vi "Right Click.vi"(6 "Empty Line?":bool, 7 "object refs":T2, 8 "error in (no error)":errorcluster, 9 "Coords":T1, 10 "Event data":variant, 11 "Multi Column Listbox in":refnum<class "Multi Column Listbox.lvclass">) -> (0 "error out":errorcluster, 3 "Multi Column Listbox out":refnum<class "Multi Column Listbox.lvclass">)   [LabVIEW 2014, in "Table Manager.lvlib" / "Multi Column Listbox.lvclass"]
doc: "Displays the menu options on a Right-Click."
uses:
  Multi Column Listbox.lvclass
  Table Manager/object ref.ctl
  Configuration Editor/Classes/Engine Parent/Engine Parent Editor Node.lvclass
  Configuration Editor/Classes/Module editor node/module editor node.lvclass
  <vilib>/Utility/miscctls.llb/LVPoint32TypeDef.ctl
  Multi Column Listbox.lvclass/Multi Column Listbox.ctl
  Table Manager/Menu Options.ctl
  <vilib>/NI/Tag Bus/tag/tag descriptor.lvclass
  Table Manager.lvlib
  <vilib>/NI/Tag Bus Module Framework/module configuration/TBM module configuration.lvclass
  Table Manager/Table Manager.lvclass
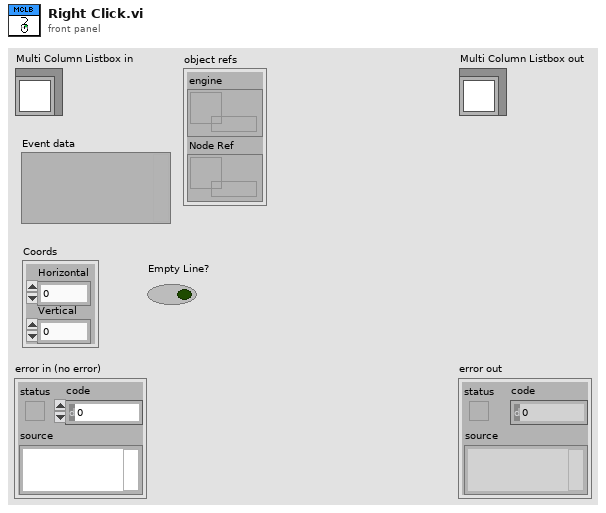
[diagram p1: front panel]
types:
  T1 = typedef "LVPoint32TypeDef.ctl" = cluster{"Horizontal":i32, "Vertical":i32}
  T2 = typedef "Table Manager.lvlib/Table Manager.lvclass/object ref.ctl" = cluster{"engine":refnum<data-value>, "Node Ref":refnum<data-value>}
  T3 = typedef "LVRowAndColumnTypeDef.ctl" = cluster{"Row":i32, "Column":i32}
  T4 = typedef "Table Manager.lvlib/Table Manager.lvclass/Menu Options.ctl" = enum16{"Always Show", "Show When Used", "Show When Empty"}
  T5 = typedef "Table Manager.lvlib/Table Manager.lvclass/Menu Definition.ctl" = cluster{"Menu Name":string, "Menu Options":T4}
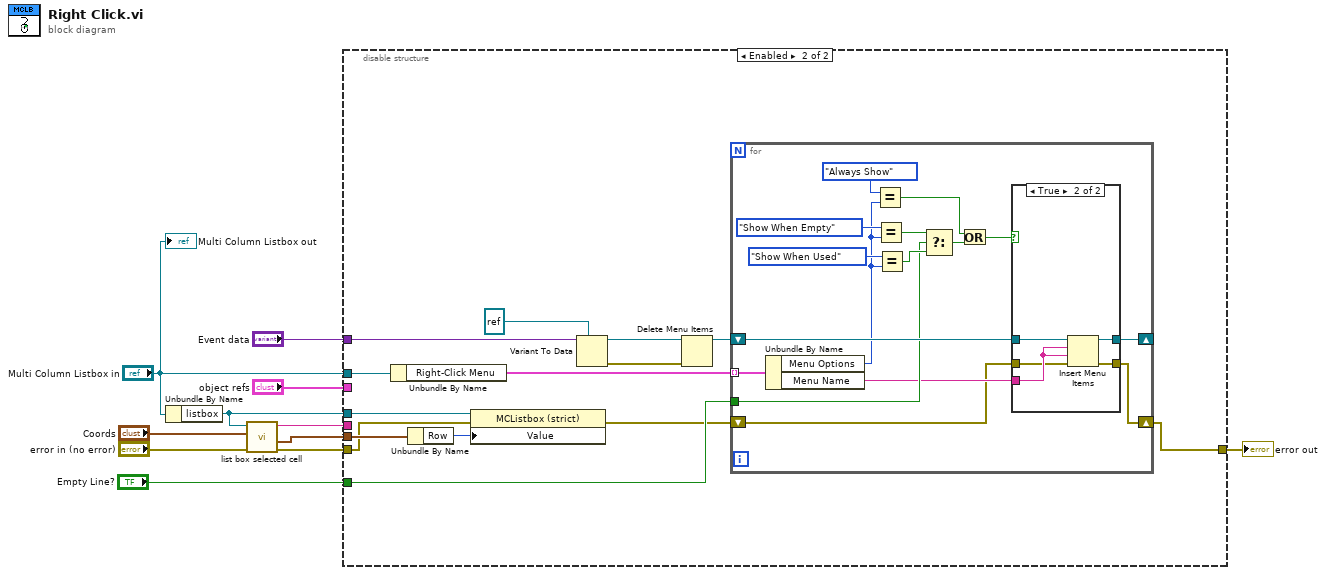
[diagram p0: block diagram]
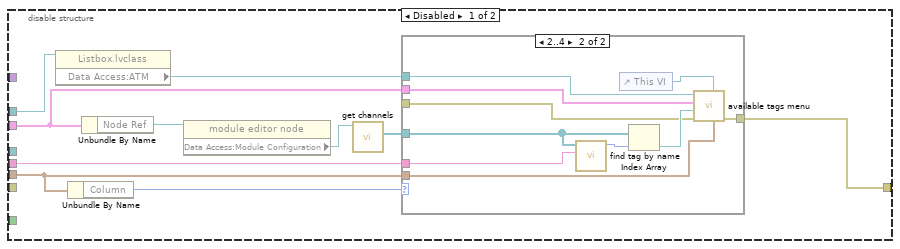
[diagram p2: hidden frame]
diagram:
  n1 = Unbundle By Name("Multi Column Listbox in") -> ("listbox"=w3:refnum<vi>)
  n2 = call "list box selected cell.vi"("error in"="error in (no error)", "Coords"="Coords", "MulticolumnListbox in"=w3) -> ("error out"=w5:errorcluster, "cell position"=w6:T3, "tag select name"=w7:string)  [unwired: 5 in, 1 out]
  n3 = disable-structure shown="Enabled" {
    disable-tunnel: "object refs" -> [w17 _]
    disable-tunnel: [w16 w33] -> w10
    disable-tunnel: "Multi Column Listbox in" -> [w15 w42]
    disable-tunnel: "Event data" -> [_ w46]
    disable-tunnel: w7 -> [w13 _]
    disable-tunnel: w6 -> [w12 w38]
    disable-tunnel: w5 -> [_ w35]
    disable-tunnel: w3 -> [_ w39]
    disable-tunnel: "Empty Line?" -> [_ w36]
    frame Disabled {
      n4 = property class="Listbox.lvclass"(reference=w15) -> ("Data Access:ATM"=w14:refnum<user-event>)  [unwired: 1 in, 2 out]
      n5 = Unbundle By Name(w12) -> ("Column"=w19:i32)
      n6 = Unbundle By Name(w17) -> ("Node Ref"=w18:refnum<data-value>)
      n7 = property class="module editor node"(reference=w18) -> ("Data Access:Module Configuration"=w21:refnum<class "TBM module configuration.lvclass">)  [unwired: 1 in, 2 out]
      n8 = call-dynamic "get channels.vi"("module configuration in"=w21) -> ("channels"=w20:refnum<class "TBM channel.lvclass">[])  [unwired: 9 in, 1 out]
      n9 = case shown="2..4" w19 {
        tunnel: w20 -> [_ w31]
        tunnel: w13 -> [_ w30]
        tunnel: w14 -> [_ w27]
        tunnel: w17 -> [_ w26]
        tunnel: [w22 w25] -> w16
        tunnel: _ -> [w22 w24]
        tunnel: w12 -> [_ w23]
        frame 0, Default {
        }
        frame 2..4 {
          n10 = call <vilib>:"find tag by name.vi"("name"=w30, "tags in"=w31) -> ("index"=w32:i32)  [unwired: 9 in]
          n11 = control-ref of="This VI"() -> (w29:refnum<vi>)
          n12 = Index Array(array=w31, index=w32) -> (element=w28:refnum<class "TBM channel.lvclass">)
          n13 = call "available tags menu.vi"("Point32"=w23, "parent vi reference"=w29, "error in"=w24, "channel to map to"=w28, "object ref"=w26, "ATM"=w27) -> ("error out"=w25:errorcluster)  [unwired: 5 in]
        }
      }
    }
    frame Enabled {
      n14 = Unbundle By Name(w42) -> ("Right-Click Menu"=w41:T5[])
      n15 = Unbundle By Name(w38) -> ("Row"=w37:i32)
      n16 = property class="MCListbox (strict)"(reference=w39, error in=w35, "Value"=w37) -> (error out=w34:errorcluster)  [unwired: 1 out]
      n17 = Variant To Data(type=refnum<k9> refnum ("MenuRef"), Variant=w46) -> (data=w44:refnum<k9>, error out=w43:errorcluster)  [unwired: 1 in]
      n18 = Delete Menu Items(6:w43, 9:w44) -> (3:w40:refnum<k9>)  [unwired: 2 in, 1 out]
      n19 = for {
        tunnel: w41 -> [w60] mode=indexing
        shift-right: [w61] -> _
        shift-left: w40 -> [w62]
        tunnel: w36 -> [w53]
        shift-right: [w47] -> w33
        shift-left: w34 -> [w48]
        n20 = Unbundle By Name(w60) -> ("Menu Options"=w56:T4, "Menu Name"=w49:string)
        n21 = Equal?(x=Menu_Options."Always Show" ("y"), y=w56) -> (x = y?=w51:bool)
        n22 = Equal?(x=Menu_Options."Show When Empty" ("y"), y=w56) -> (x = y?=w55:bool)
        n23 = Equal?(x=Menu_Options."Show When Used" ("y"), y=w56) -> (x = y?=w54:bool)
        n24 = Select(t=w55, s=w53, f=w54) -> (s? t:f=w52:bool)
        n25 = Or(x=w51, y=w52) -> (x .or. y?=w50:bool)
        n26 = case shown="True" w50 {
          tunnel: w62 -> [w64 w69]
          tunnel: [w64 w68] -> w61
          tunnel: w49 -> [_ w67]
          tunnel: w48 -> [w63 w66]
          tunnel: [w63 w65] -> w47
          frame False {
          }
          frame True {
            n27 = Insert Menu Items(6:w66, 7:w67, 8:w67, 9:w69) -> (0:w65:errorcluster, 3:w68:refnum<k9>)  [unwired: 2 in, 1 out]
          }
        }
      }
    }
  }
  "error out" <- w10
  "Multi Column Listbox out" <- "Multi Column Listbox in"
